vi "MQTT Properties - Decode.vi"(7 "Encoded MQTT Properties":u8[](array[numeric]), 11 "error in (no error)":errorcluster) -> (4 "remaining data":u8[](array[numeric]), 8 "MQTT Properties":T1[](array[typedef]) {"Property" items=["Payload Format Indicator"=1, "Message Expiry Interval"=2, "Content Type"=3, "Response Topic"=8, "Correlation Data"=9, "Subscription Identifier"=11, "Session Expiry Interval"=17, "Assigned Client Identifier"=18, "Server Keep Alive"=19, "Authentication Method"=21, "Authentication Data"=22, "Request Problem Information"=23, "Will Delay Interval"=24, "Request Response Information"=25, "Response Information"=26, "Server Reference"=28, "Reason String"=31, "Receive Maximum"=33, "Topic Alias Maximum"=34, "Topic Alias"=35, "Maximum QoS"=36, "Retain Available"=37, "User Property"=38, "Maximum Packet Size"=39, "Wildcard Subscription Available"=40, "Subscription Identifier Available"=41, "Shared Subscription Available"=42]}, 15 "error out":errorcluster)   [LabVIEW 2019, in "KoRE-MQTT.lvlib"]
doc: "Copyright (c) 2025 KoRElibs.com\nSPDX-License-Identifier: EUPL-1.2\n\nThis VI is licensed under the European Union Public License (EUPL) Version 1.2. You may use this VI unmodified in proprietary works. If you distribute a modified version of this file, the modified file must be released under the EUPL-1.2. Full license: https://joinup.ec.europa.eu/asset/eupl/eupl/1.2/"
uses:
  KoRE-MQTT.lvlib
  Public/TypeDefs/MQTT Property - GENERIC.ctl
  Public/TypeDefs/MQTT Property Type.ctl
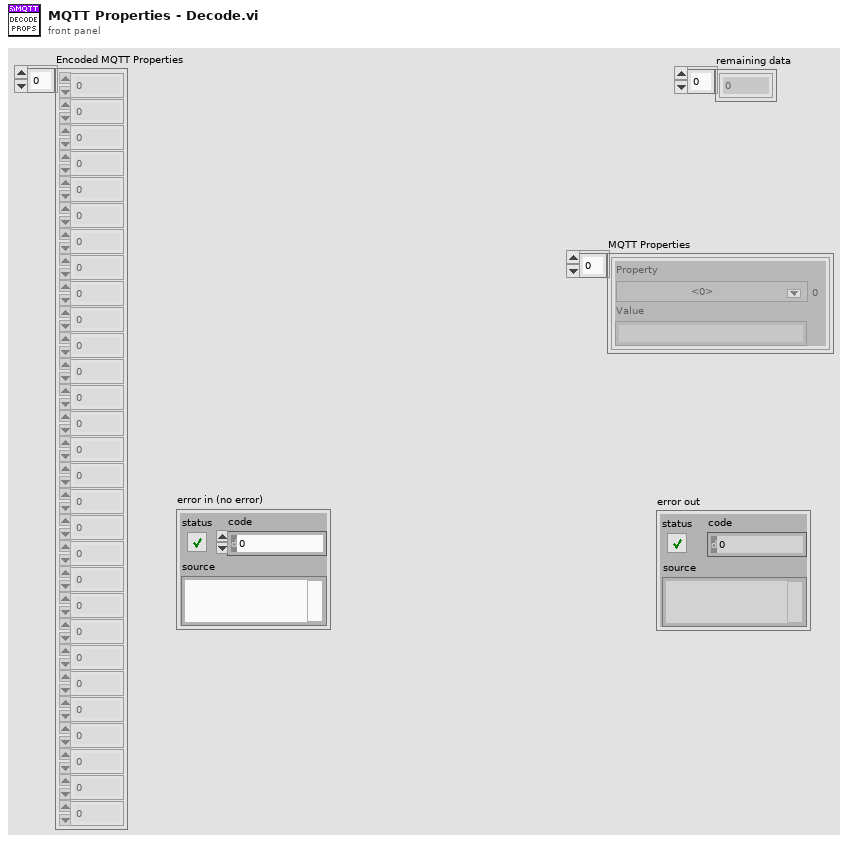
[diagram p1: front panel]
types:
  T1 = typedef "KoRE-MQTT.lvlib/MQTT Property - GENERIC.ctl" = cluster{"Property":T2, "Value":string}
  T2 = typedef "KoRE-MQTT.lvlib/MQTT Property Type.ctl" = u8
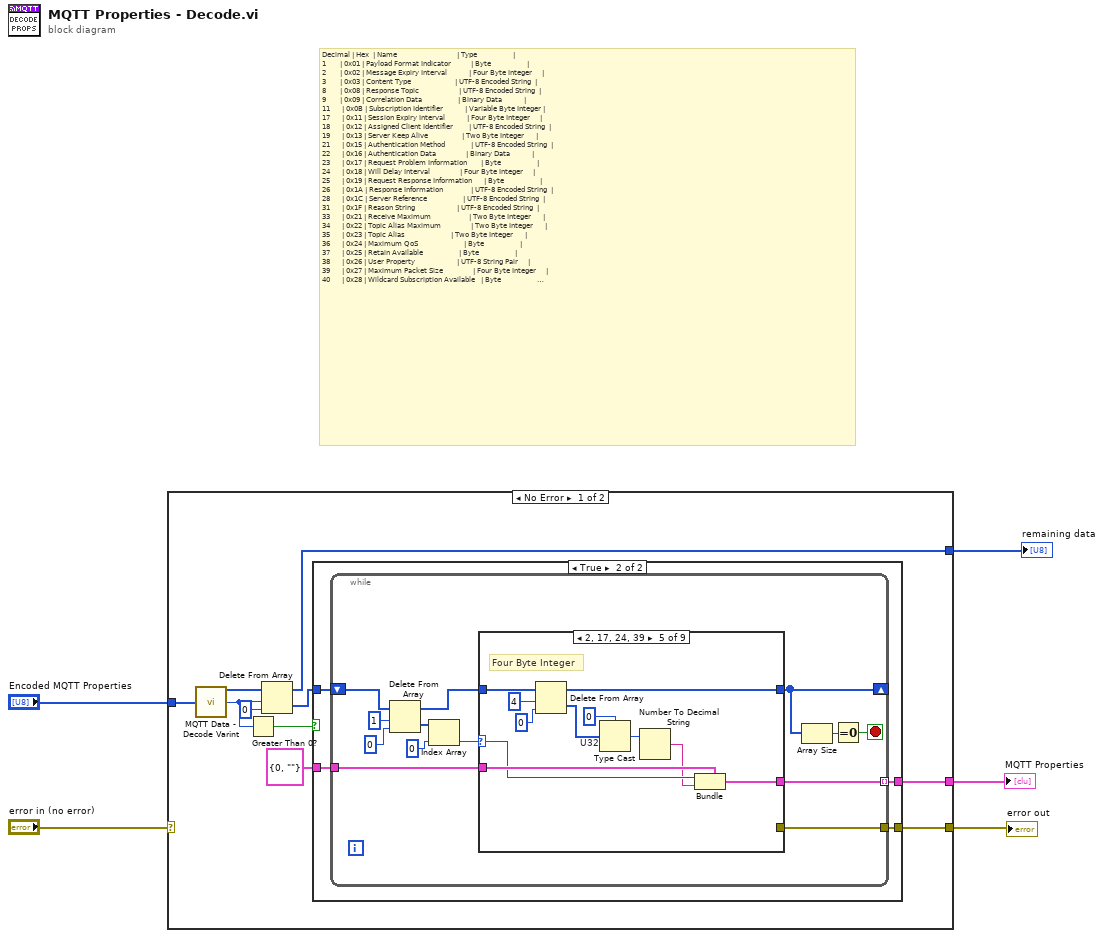
[diagram p0: block diagram]
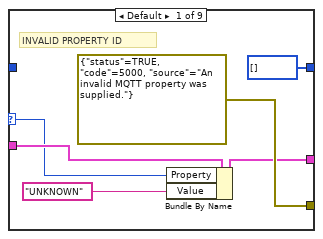
[diagram p3: hidden frame]
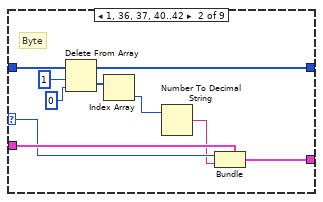
[diagram p4: hidden frame]
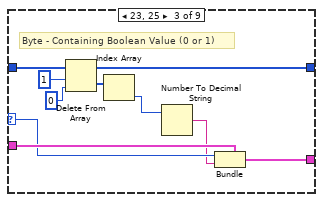
[diagram p5: hidden frame]
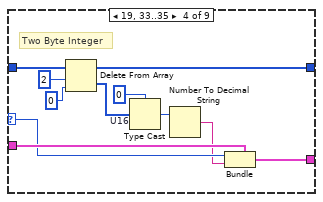
[diagram p6: hidden frame]
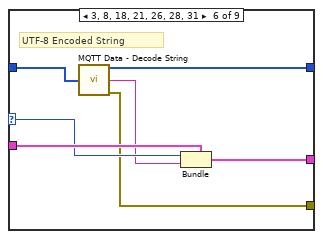
[diagram p7: hidden frame]
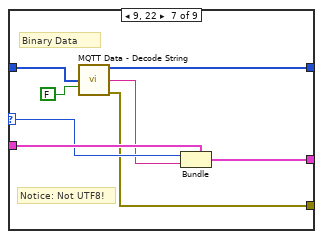
[diagram p8: hidden frame]
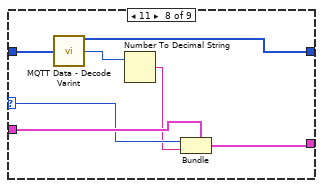
[diagram p9: hidden frame]
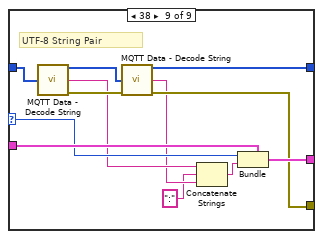
[diagram p10: hidden frame]
diagram:
  # "Decimal | Hex  | Name                              | Type                  |\n1       | 0x01 | Payload Format Indicator          | Byte                  |\n2       | 0x02 | Message Expiry Interval           | Four Byte Integer     |\n3       | 0x03 | Content Type                      | UTF-8 Encoded String  |\n8       | 0x08 | Response Topic                    | UTF-8 Encoded String  |\n9       | 0x09 | Correlation Data                  | Binary Data           |\n11      | 0x0B | Subscription Identifier           | Variable Byte Integer |\n17      | 0x11 | Session Expiry Interval           | Four Byte Integer     |\n18      | 0x12 | Assigned Client Identifier        | UTF-8 Encoded String  |\n19      | 0x13 | Server Keep Alive                 | Two Byte Integer      |\n21      | 0x15 | Authentication Method             | UTF-8 Encoded String  |\n22      | 0x16 | Authentication Data               | Binary Data           |\n23      | 0x17 | Request Problem Information       | Byte                  |\n24      | 0x18 | Will Delay Interval               | Four Byte Integer     |\n25      | 0x19 | Request Response Information      | Byte                  |\n26      | 0x1A | Response Information              | UTF-8 Encoded String  |\n28      | 0x1C | Server Reference                  | UTF-8 Encoded String  |\n31      | 0x1F | Reason String                     | UTF-8 Encoded String  |\n33      | 0x21 | Receive Maximum                   | Two Byte Integer      |\n34      | 0x22 | Topic Alias Maximum               | Two Byte Integer      |\n35      | 0x23 | Topic Alias                       | Two Byte Integer      |\n36      | 0x24 | Maximum QoS                       | Byte                  |\n37      | 0x25 | Retain Available                  | Byte                  |\n38      | 0x26 | User Property                     | UTF-8 String Pair     |\n39      | 0x27 | Maximum Packet Size               | Four Byte Integer     |\n40      | 0x28 | Wildcard Subscription Available   | Byte                  |\n41      | 0x29 | Subscription Identifier Available | Byte                  |\n42      | 0x2A | Shared Subscription Available     | Byte                  |"
  n1 = case shown="No Error" "error in (no error)" {
    selector: "error in (no error)" -> [_ w115]
    tunnel: "Encoded MQTT Properties" -> [w15 _]
    tunnel: [w13 _] -> w4
    tunnel: [w12 w115] -> w3
    tunnel: [w9 _] -> w2
    frame No Error {
      n2 = call "MQTT Data - Decode Varint.vi"("Variable Length Integer Data"=w15) -> ("remaining data"=w11:u8[], "Value"=w8:i32)  [unwired: 12 in, 1 out]
      n3 = Greater Than 0?(x=w8) -> (x > 0?=w7:bool)
      n4 = Delete From Array(array=w11, length=w8, index=0) -> (deleted portion=w10:u8[], array with subset deleted=w9:u8[])
      n5 = case shown="True" w7 {
        tunnel: T1 {"Property"=0, "Value"=""} ("General MQTT Property") -> [_ w19]
        tunnel: [_ w18] -> w13
        tunnel: [_ w17] -> w12
        tunnel: w10 -> [_ w16]
        frame False {
        }
        frame True {
          n6 = while {
            shift-right: [w23] -> _
            shift-left: w16 -> [w32]
            tunnel: w19 -> [w31]
            tunnel: [w30] -> w18 mode=indexing
            tunnel: [w22] -> w17
            stop <- w20 stop-if-true
            n7 = Delete From Array(array=w32, length=1, index=0) -> (deleted portion=w27:u8[], array with subset deleted=w24:u8[])
            n8 = Index Array(array=w27, index=0) -> (element=w25:u8)
            n9 = case shown="2, 17, 24, 39" w25 {
              selector: w25 -> [w34 w47 w57 w68 w79 w84 w92 w99 w112]
              tunnel: w24 -> [_ w46 w56 w67 w78 w87 w95 w102 w114]
              tunnel: w31 -> [w36 w48 w58 w69 w80 w85 w93 w100 w113]
              tunnel: [u8[] [] ("remaining data") w43 w53 w64 w75 w86 w94 w101 w109] -> w23
              tunnel: [w35 w39 w49 w62 w73 w82 w90 w96 w111] -> w30
              tunnel: [errorcluster {"status"=TRUE, "code"=5000, "source"="An invalid MQTT property was supplied."} ("error out") _ _ _ _ w81 w89 _ w107] -> w22
              frame Default {
                # "INVALID PROPERTY ID"
                n10 = Bundle By Name(cluster=w36, "Property"=w34, "Value"="UNKNOWN") -> (w35:T1)
              }
              frame 1, 36, 37, 40..42 {
                # "Byte"
                n11 = Delete From Array(array=w46, length=1, index=0) -> (deleted portion=w42:u8[], array with subset deleted=w43:u8[])
                n12 = Index Array(array=w42) -> (element=w41:u8)  [unwired: 1 in]
                n13 = Number To Decimal String(number=w41) -> (decimal integer string=w40:string)  [unwired: 1 in]
                n14 = Bundle(cluster=w48, "Property"=w47, "Value"=w40) -> (w39:T1)
              }
              frame 23, 25 {
                # "Byte - Containing Boolean Value (0 or 1)"
                n15 = Delete From Array(array=w56, length=1, index=0) -> (deleted portion=w52:u8[], array with subset deleted=w53:u8[])
                n16 = Index Array(array=w52) -> (element=w51:u8)  [unwired: 1 in]
                n17 = Number To Decimal String(number=w51) -> (decimal integer string=w50:string)  [unwired: 1 in]
                n18 = Bundle(cluster=w58, "Property"=w57, "Value"=w50) -> (w49:T1)
              }
              frame 19, 33..35 {
                w60 = u16 0  # U16
                # "Two Byte Integer"
                n19 = Delete From Array(array=w67, length=2, index=0) -> (deleted portion=w61:u8[], array with subset deleted=w64:u8[])
                n20 = Type Cast(type=w60, x=w61) -> (*(type *) &x=w59:u16)
                n21 = Number To Decimal String(number=w59) -> (decimal integer string=w63:string)  [unwired: 1 in]
                n22 = Bundle(cluster=w69, "Property"=w68, "Value"=w63) -> (w62:T1)
              }
              frame 2, 17, 24, 39 {
                w71 = u32 0  # U32
                # "Four Byte Integer"
                n23 = Delete From Array(array=w78, length=4, index=0) -> (deleted portion=w72:u8[], array with subset deleted=w75:u8[])
                n24 = Type Cast(type=w71, x=w72) -> (*(type *) &x=w70:u32)
                n25 = Number To Decimal String(number=w70) -> (decimal integer string=w74:string)  [unwired: 1 in]
                n26 = Bundle(cluster=w80, "Property"=w79, "Value"=w74) -> (w73:T1)
              }
              frame 3, 8, 18, 21, 26, 28, 31 {
                # "UTF-8 Encoded String"
                n27 = call "MQTT Data - Decode String.vi"("Encoded String"=w87) -> ("remaining data"=w86:u8[], "String"=w83:string, "error out"=w81:errorcluster)  [unwired: 12 in]
                n28 = Bundle(cluster=w85, "Property"=w84, "Value"=w83) -> (w82:T1)
              }
              frame 9, 22 {
                # "Notice: Not UTF8!"
                # "Binary Data"
                n29 = call "MQTT Data - Decode String.vi"("Encoded String"=w95, "From UTF8?"=FALSE) -> ("remaining data"=w94:u8[], "String"=w91:string, "error out"=w89:errorcluster)  [unwired: 11 in]
                n30 = Bundle(cluster=w93, "Property"=w92, "Value"=w91) -> (w90:T1)
              }
              frame 11 {
                n31 = call "MQTT Data - Decode Varint.vi"("Variable Length Integer Data"=w102) -> ("remaining data"=w101:u8[], "Value"=w98:i32)  [unwired: 12 in, 1 out]
                n32 = Number To Decimal String(number=w98) -> (decimal integer string=w97:string)  [unwired: 1 in]
                n33 = Bundle(cluster=w100, "Property"=w99, "Value"=w97) -> (w96:T1)
              }
              frame 38 {
                # "UTF-8 String Pair"
                n34 = call "MQTT Data - Decode String.vi"("Encoded String"=w114) -> ("remaining data"=w110:u8[], "String"=w106:string, "error out"=w108:errorcluster)  [unwired: 12 in]
                n35 = call "MQTT Data - Decode String.vi"("Encoded String"=w110, "error in (no error)"=w108) -> ("remaining data"=w109:u8[], "String"=w105:string, "error out"=w107:errorcluster)  [unwired: 11 in]
                n36 = Concatenate Strings(w106, ":" ("element"), w105) -> (w103:string)
                n37 = Bundle(cluster=w113, "Property"=w112, "Value"=w103) -> (w111:T1)
              }
            }
            n38 = Array Size(array=w23) -> (size(s)=w21:i32)
            n39 = Equal To 0?(x=w21) -> (x = 0?=w20:bool)
          }
        }
      }
    }
    frame Error {
    }
  }
  "MQTT Properties" <- w4
  "error out" <- w3
  "remaining data" <- w2
